vi "VIH ExtCmd - Check VIHRUN Association.vi"(8 "error in":errorcluster) -> (0 "error out":errorcluster, 2 "VIHRUN path":path, 3 "Associated":bool, 5 "In LV Folder":bool, 7 "Implemented":bool)   [LabVIEW 2014]
doc: "::: VI Helpeks :::\nCopyright (c) 2000-2026 Konstantin Shifershteyn. All rights reserved."
uses:
  <vilib>/registry/registry.llb/Registry RtKey.ctl
  <vilib>/registry/registry.llb/Registry SAM.ctl
  <vilib>/registry/registry.llb/Read Registry Value Simple STR.vi
panel:
  # "VI Helpeks\nCopyright (c) 2012-2026 Konstantin Shifershteyn"
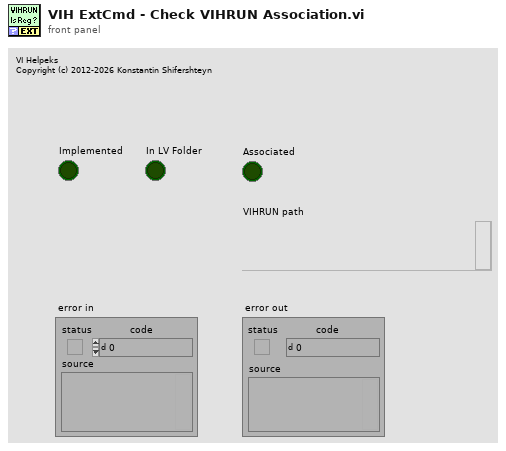
[diagram p1: front panel]
types:
  T1 = typedef "Registry SAM.ctl" = enum32{"KEY_QUERY_VALUE", "KEY_SET_VALUE", "KEY_CREATE_SUB_KEY", "KEY_ENUMERATE_SUB_KEYS", "KEY_NOTIFY", "KEY_CREATE_LINK", "KEY_READ", "KEY_WRITE", "KEY_ALL_ACCESS", "KEY_READ | KEY_WRITE"}
  T2 = typedef "Registry RtKey.ctl" = enum32{"HKEY_CLASSES_ROOT", "HKEY_CURRENT_USER", "HKEY_LOCAL_MACHINE", "HKEY_USERS", "HKEY_PERFORMANCE_DATA", "HKEY_CURRENT_CONFIG", "HKEY_DYN_DATA"}
  T3 = cluster{"Product Name":string, "Short Name":string, "Product Version":string, "Release Timestamp":string, "Developer":string, "Copyright":string}
  T4 = cluster{"Extension":string, "Program ID":string, "DefaultIcon":string, "OpenCommand":string}
  T5 = typedef "Registry refnum.ctl" = refnum<k1>
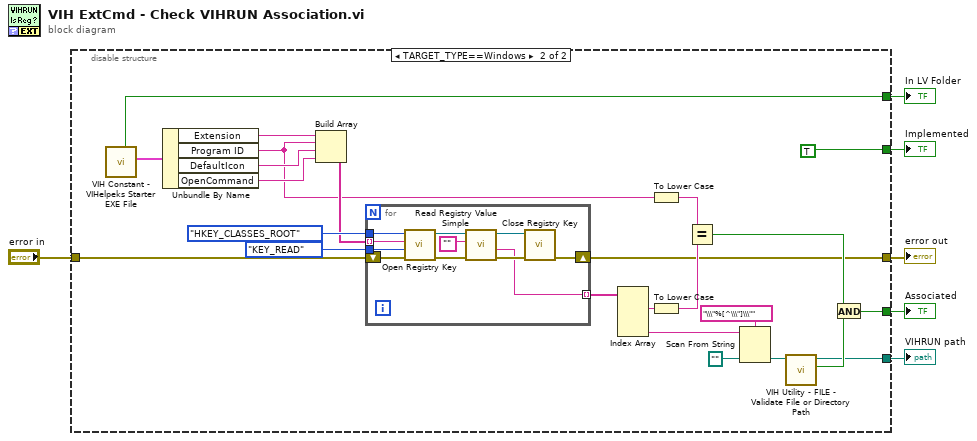
[diagram p0: block diagram]
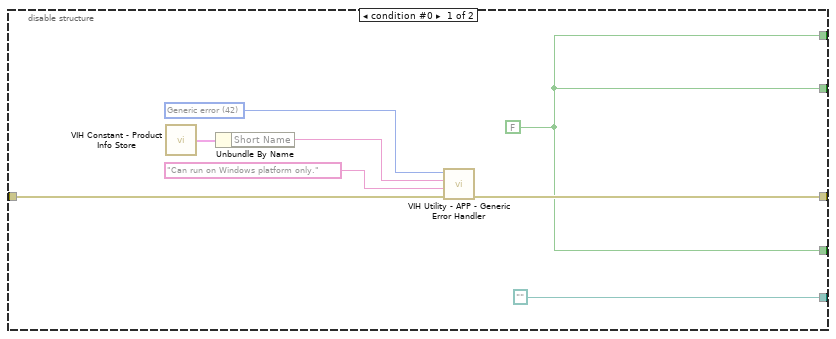
[diagram p2: hidden frame]
diagram:
  n1 = disable-structure shown="TARGET_TYPE==Windows" {
    disable-tunnel: [w7 w28] -> w6
    disable-tunnel: [path "" w27] -> w5
    disable-tunnel: [w7 w18] -> w4
    disable-tunnel: [w8 w17] -> w3
    disable-tunnel: "error in" -> [w9 w16]
    disable-tunnel: [w7 TRUE] -> w1
    frame condition #0 {
      w10 = 42 items=["No error", "Argument error", "Memory is full", "Out of zone", "End of file", "File already open", "Generic file I/O error", "File not found", "File permission error", "Disk is full", "Duplicate path", "Too many files open", "System feature not enabled", "Resource file not found", "Cannot add resource", "Resource not found", "Image not found", "Image memory error", "Pen does not exist", "Config type invalid", "Config token not found", "Config parse error", "Config memory error", "Bad external code format", "Bad external code offset", "External code not present", "Null window", "Destroy window error", "Null menu", "Print aborted", "Bad print record", "Print driver error", "Windows error during printing", "Memory error during printing", "Print dialog error", "Generic print error", "Invalid device refnum", "Device not found", "Device parameter error", "Device unit error", "Cannot open device", "Device call aborted", "Generic error", "Cancelled by user", "Object ID too low", "Object ID too high", "Object not in heap", "Unknown heap", "Unknown object (invalid DefProc)", "Unknown object (DefProc not in table)", "Message out of range", "Invalid (null) method", "Unknown message", "Manager call not supported", "Bad address", "Network operation in progress", "Network operation timed out", "Connection is busy", "Network attribute not supported", "Network error", "Address in use", "System out of memory", "Connection aborted", "Connection refused", "Not connected", "Already connected", "Connection closed", "Initialization error (interapplication manager)", "Bad occurrence", "Wait on unbound occurrence handler", "Occurrence queue overflow", "Datalog type conflict", "Unused", "Unrecognized type (interapplication manager)", "Memory corrupt", "Failed to make temporary DLL", "Old CIN version", "Drag socket not found", "Failed to load drop-object", "Failed to register OLE object", "Failed to release OLE object", "Format specifier type mismatch", "Unknown format specifier", "Too few format specifiers", "Too many format specifiers", "Scan failed", "Newer CIN version", "Error converting to variant", "Runtime menu error", "Password tampered", "Variant attribute not found", "Incompatible variant data type", "Event data is not available", "Event Store is not present", "Occurrence is not found", "Event Queue is not created", "Event info is not available in the type library", "Refnum passed is NULL", "Error retrieving Class GUID", "Error retrieving CoClass GUID", "Error retrieving TypeLib GUID.", "Bad built application magic bytes.", "Specific driver is different from the specific driver associated with the Logical Name.", "There is no session opened to the class driver.", "Max Error", "MAX - Error with config objects", "MAX - Error loading configuration", "MAX - Group not supported", "Singlecast connections can not send to multicast addresses.", "Multicast connections can not send to singlecast addresses.", "Specified IP address not in multicast address range.", "Attempt to write to read-only multicast connection.", "Attempt to read from write-only multicast connection.", "The buffer used to receive a datagram was smaller than the datagram itself"]
      w7 = FALSE
      n2 = call "VIH Constant - Product Info Store.vi"() -> ("Product Info"=w12:T3)
      n3 = Unbundle By Name(w12) -> ("Short Name"=w13:string)
      n4 = call "VIH Utility - APP - Generic Error Handler.vi"("error in"=w9, "error reason"="Can run on Windows platform only.", "error location"=w13, "error code"=w10) -> ("error out"=w8:errorcluster)  [unwired: 6 in, 1 out]
    }
    frame condition #1 (active) {
      n5 = call "VIH Constant - VIHelpeks Starter EXE File.vi"() -> ("Registry Keys"=w26:T4, "In LV Folder"=w18:bool)  [unwired: 9 in, 1 out]
      n6 = Unbundle By Name(w26) -> ("Extension"=w25:string, "Program ID"=w20:string, "DefaultIcon"=w24:string, "OpenCommand"=w23:string)
      n7 = Build Array(w25, w20, w24, w23) -> (w22:string[])
      n8 = for {
        tunnel: Registry_RtKey."HKEY_CLASSES_ROOT" ("root key (HKEY_LOCAL_MACHINE)") -> [w49]
        tunnel: Registry_SAM."KEY_READ" ("security access mask (KEY_READ | KEY_WRITE)") -> [w48]
        tunnel: w22 -> [w42] mode=indexing
        tunnel: [w41] -> w33 mode=indexing
        shift-right: [w40] -> w17
        shift-left: w16 -> [w39]
        n9 = call <vilib>:"Open Registry Key.vi"("error in (no error)"=w39, "security access mask (KEY_READ | KEY_WRITE)"=w48, "subkey"=w42, "root key (HKEY_LOCAL_MACHINE)"=w49) -> ("error out"=w46:errorcluster, "refnum out"=w47:T5)  [unwired: 6 in]
        n10 = call-poly <vilib>:"Read Registry Value Simple.vi"("error in (no error)"=w46, "value"="", "refnum"=w47) -> ("error out"=w44:errorcluster, "String/Binary data"=w41:string, "refnum out"=w45:T5)  [unwired: 3 in, 1 out]
        n11 = call <vilib>:"Close Registry Key.vi"("error in (no error)"=w44, "refnum"=w45) -> ("error out"=w40:errorcluster)  [unwired: 5 in]
      }
      n12 = Index Array(array=w33) -> (element #1=w21:string, element #4=w19:string)  [unwired: 4 in, 2 out]
      n13 = To Lower Case(string=w20) -> (all lower case string=w31:string)
      n14 = To Lower Case(string=w21) -> (all lower case string=w30:string)
      n15 = Equal?(x=w31, y=w30) -> (x = y?=w32:bool)
      n16 = Scan From String(format string="\\\"%[^\\\"]\\\"", input string=w19, default 1=path "") -> (output 1=w34:path)  [unwired: 2 in, 3 out]
      n17 = call "VIH Utility - FILE - Validate File or Directory Path.vi"("Path"=w34) -> ("file"=w29:bool, "dup Path"=w27:path)  [unwired: 6 in, 3 out]
      n18 = And(x=w32, y=w29) -> (x .and. y?=w28:bool)
    }
  }
  "Associated" <- w6
  "VIHRUN path" <- w5
  "In LV Folder" <- w4
  "error out" <- w3
  "Implemented" <- w1
